vi "Wifi USRP Receiver with Queue.vi"() -> ()   [LabVIEW 2024]
uses:
  <vilib>/Analysis/2dsp.llb/Inverse Complex FFT.vi
  <vilib>/Analysis/2dsp.llb/Complex FFT.vi
  <vilib>/addons/Modulation/Digital/Support/Common/Validators/mod_Validate Number of Rows Columns.vi
  <vilib>/addons/Modulation/Digital/Channel Coding/Block codes/subVIs/mod_Buffer block code info.vi
  <vilib>/addons/Modulation/Digital/DeInterleaving/Block DeInterleaver/mod_Block DeInterleaver (Matrix).vi
  <vilib>/addons/Modulation/Digital/Support/Common/Validators/mod_Generate Bits Validate.vi
  <vilib>/addons/Modulation/Digital/General/subVIs/mod_Generate Bits Pattern.vi
  <vilib>/addons/Modulation/Analog/support/mod_Set Error Source.vi
  <vilib>/addons/Modulation/Digital/General/MT Map PSK Symbols to Bits.vi
  <vilib>/addons/Modulation/Digital/Channel Coding/MT Convolutional Decoder (Viterbi Hard Decision, Rate).vi
  <vilib>/addons/Modulation/Digital/General/MT Map QAM Symbols to Bits.vi
  <vilib>/addons/Modulation/Digital/General/subVIs/mod_Generate Bits PN Sequence.vi
  <instrlib>/niUSRP/niUSRP Fetch Rx Data (CDB).vi
  <vilib>/Analysis/NI_AALPro.lvlib
  <vilib>/addons/Modulation/niDMT.lvlib
panel:
  out "Received Message":string
  out "Fine FO Estimation":dbl(graph)
  out "Coarse FO Estimation":dbl(graph)
  in  "Ts":dbl
  out "Plateau Length":dbl(graph)
  in  "active antenna":string
  in  "gain":dbl format="%#_6f"
  in  "carrier frequency":dbl=100000.0 format="%#_6p"
  in  "IQ rate":dbl=100000.0 format="%#_6p"
  in  "device names":refnum<k15>
  out "Data 2":dbl[](graph)
  out "Data 1":dbl[](graph)
  in  "Stop":bool
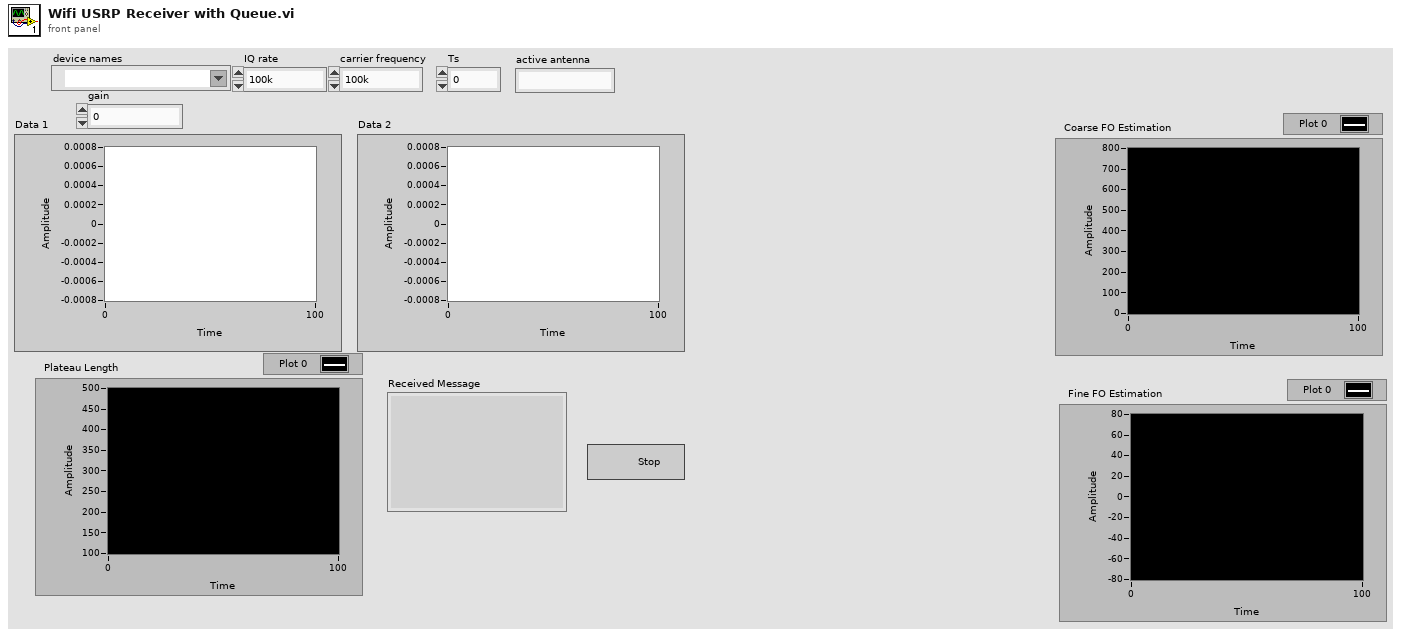
[diagram p1: front panel]
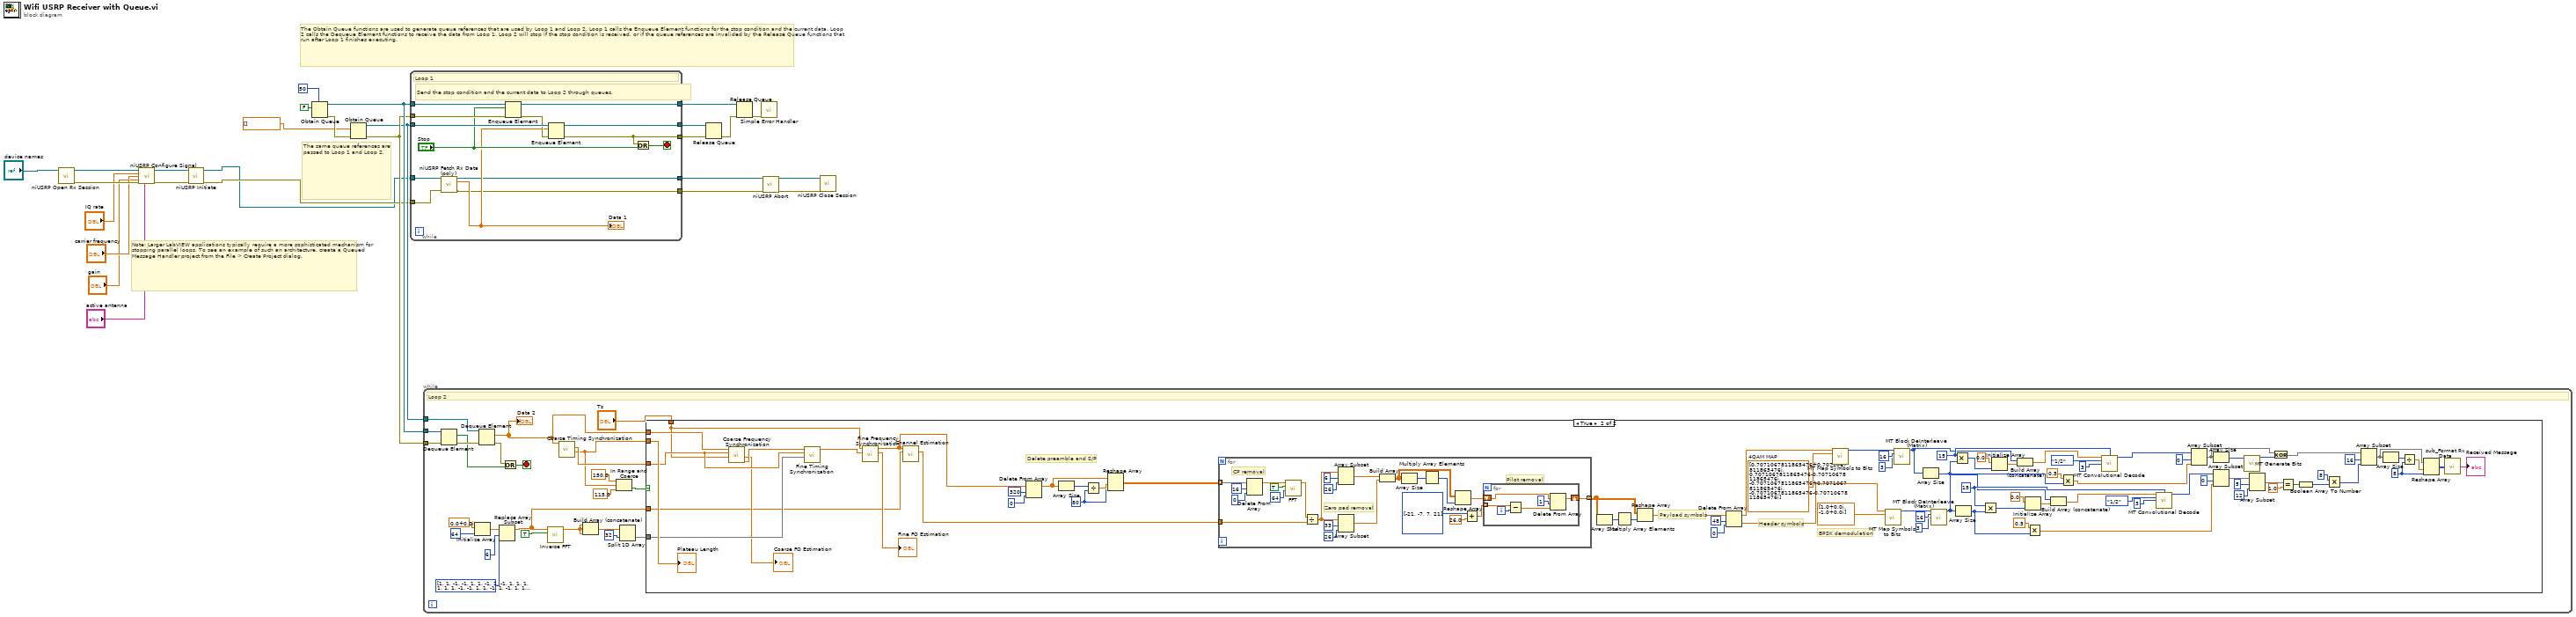
[diagram p0: block diagram]
diagram:
  # "Note: Larger LabVIEW applications typically require a more sophisticated mechanism for stopping parallel loops. To see an example of such an architecture, create a Queued Message Handler project from the File > Create Project dialog."
  # "The same queue references are passed to Loop 1 and Loop 2."
  # "The Obtain Queue functions are used to generate queue references that are used by Loop 1 and Loop 2. Loop 1 calls the Enqueue Element functions for the stop condition and the current data. Loop 2 calls the Dequeue Element functions to receive the data from Loop 1. Loop 2 will stop if the stop condition is received, or if the queue references are invalided by the Release Queue functions that run after Loop 1 finishes executing."
  n1 = call <instrlib>:"niUSRP Open Rx Session.vi"("device names"="device names") -> ("session handle out"=w16:refnum<k15>, "error out"=w14:errorcluster)  [unwired: 13 in]
  n2 = call <instrlib>:"niUSRP Configure Signal.vi"("session handle"=w16, "IQ rate"="IQ rate", "carrier frequency"="carrier frequency", "gain"="gain", "error in (no error)"=w14, "active antenna"="active antenna") -> ("session handle out"=w15:refnum<k15>, "error out"=w13:errorcluster)  [unwired: 5 in, 3 out]
  n3 = call <instrlib>:"niUSRP Initiate.vi"("session handle"=w15, "error in (no error)"=w13) -> ("session handle out"=w6:refnum<k15>, "error out"=w7:errorcluster)  [unwired: 12 in]
  n4 = Obtain Queue(max queue size (-1, unlimited)=50, element data type=FALSE) -> (queue out=w27:refnum<queue>, error out=w25:errorcluster)  [unwired: 3 in, 1 out]
  n5 = Obtain Queue(element data type=cdb[] [], error in (no error)=w25) -> (queue out=w18:refnum<queue>, error out=w19:errorcluster)  [unwired: 3 in, 1 out]
  n6 = while {
    tunnel: w27 -> [w41]
    tunnel: w19 -> [w40]
    tunnel: [w39] -> w21
    tunnel: w18 -> [w38]
    tunnel: [w36] -> w23
    tunnel: [w35] -> w24
    tunnel: w7 -> [w32]
    tunnel: w6 -> [w31]
    tunnel: [w29] -> w3
    tunnel: [w28] -> w2
    stop <- w33 stop-if-true
    # "Send the stop condition and the current data to Loop 2 through queues."
    # "Loop 1"
    n7 = call-poly <instrlib>:"niUSRP Fetch Rx Data (poly).vi"("session handle"=w31, "error in (no error)"=w32) -> ("session handle out"=w28:refnum<k15>, "data"=w30:cdb[], "error out"=w29:errorcluster)  [unwired: 10 in, 1 out]
    "Data 1" <- w30
    n8 = Enqueue Element(queue=w41, element="Stop", error in (no error)=w40) -> (queue out=w39:refnum<queue>, error out=w37:errorcluster)  [unwired: 1 in, 1 out]
    n9 = Enqueue Element(queue=w38, element=w30, error in (no error)=w37) -> (queue out=w36:refnum<queue>, error out=w35:errorcluster)  [unwired: 1 in, 1 out]
    n10 = Or(x=w35, y="Stop") -> (x .or. y?=w33:bool)
  }
  n11 = while {
    tunnel: w27 -> [w65]
    tunnel: w19 -> [w66]
    tunnel: w18 -> [w63]
    stop <- w60 stop-if-true
    # "Loop 2"
    n12 = Dequeue Element(queue=w65, error in (no error)=w66) -> (element=w61:bool, error out=w64:errorcluster)  [unwired: 1 in, 2 out]
    n13 = Initialize Array(cdb 0.0+0.0i ("element"), 64 ("dimension size")) -> (w54:cdb[])
    n14 = Dequeue Element(queue=w63, error in (no error)=w64) -> (element=w57:cdb[], error out=w62:errorcluster)  [unwired: 1 in, 2 out]
    "Data 2" <- w57
    n15 = Replace Array Subset(array=w54, new element=i32[] [1, 1, -1, -1, 1, 1, -1, 1, -1, 1, 1, 1, 1, 1, 1, -1, -1, 1, 1, -1, 1, -1, 1, 1, 1, 1, 0, 1, -1, -1, 1, 1, -1, 1, -1, 1, -1, -1, -1, -1, -1, 1, 1, -1, -1, 1, -1, 1, -1, 1, 1, 1, 1], index=6) -> (w46:cdb[])
    n16 = Or(x=w62, y=w61) -> (x .or. y?=w60:bool)
    n17 = call-poly <vilib>:"Inverse FFT.vi"("shift?"=TRUE ("shift? 3"), "FFT {X}"=w46) -> ("X"=w51:cdb[])  [unwired: 8 in, 1 out]
    n18 = call "Coarse Timing Synchronization.vi"("Array"=w57) -> ("max value"=w45:dbl, "Coarse packet est"=w58:dbl)  [unwired: 9 in]
    n19 = Build Array (concatenate)(w51, w51, w51) -> (w50:cdb[])
    n20 = In Range and Coerce(upper limit=150.0, x=w45, lower limit=115.0 ("y")) -> (In Range?=w42:bool)  [unwired: 1 out]
    n21 = Split 1D Array(array=w50, index=32) -> (second subarray=w47:cdb[])  [unwired: 1 out]
    n22 = case shown="True" w42 {
      tunnel: w45 -> [_ w147]
      tunnel: "Ts" -> [_ w141]
      tunnel: w58 -> [_ w144]
      tunnel: w57 -> [_ w146]
      tunnel: w47 -> [_ w143]
      tunnel: w46 -> [_ w138]
      frame False {
      }
      frame True {
        w73 = 80 ("dimension size")
        w78 = 8 ("y")
        w108 = 15 ("traceback depth (D)")
        w112 = cdb[] [0.7071067811865476+0.7071067811865476i, 0.7071067811865476-0.7071067811865476i, -0.7071067811865476+0.7071067811865476i, -0.7071067811865476-0.7071067811865476i]  # 4QAM MAP
        w120 = 15 ("traceback depth (D)")
        # "Delete preamble and S/P"
        # "Header symbols"
        # "BPSK demodulation"
        # "Payload symbols"
        n23 = call "Coarse Frequency Synchronization.vi"("Ts"=w141, "Numeric in"=w144, "Array in"=w146) -> ("Array out"=w145:cdb[], "coarse freq est"=→"Coarse FO Estimation":dbl)  [unwired: 7 in]
        n24 = call "Fine Timing Synchronization.vi"("Long Preamble"=w143, "Coarse packet est"=w144, "Frame after coarse freq sync"=w145) -> ("Frame after fine time sync"=w140:cdb[])  [unwired: 7 in, 1 out]
        n25 = call "Fine Frequency Synchronization.vi"("Frame after fine time sync"=w140, "Ts"=w141) -> ("Fine freq est"=→"Fine FO Estimation":dbl, "Frame after fine freq sync"=w67:cdb[])  [unwired: 8 in]
        n26 = call "Channel Estimation.vi"("Half of LLTF"=w138, "Frame after fine freq sync in"=w67) -> ("Channel Estimate"=w68:cdb[])  [unwired: 9 in]
        n27 = Delete From Array(array=w67, length=320, index=0) -> (array with subset deleted=w75:cdb[])  [unwired: 1 out]
        n28 = Array Size(array=w75) -> (size(s)=w72:i32)
        n29 = Divide(x=w72, y=w73) -> (x/y=w74:dbl)
        n30 = Reshape Array(w75, w74, w73) -> (w69:cdb[][])
        n31 = for {
          tunnel: w69 -> [w151] mode=indexing
          tunnel: [w153] -> w136 mode=indexing
          tunnel: w68 -> [w150]
          # "Zero pad removal"
          # "Pilot removal"
          # "CP removal"
          n32 = Delete From Array(array=w151, length=16, index=0) -> (array with subset deleted=w167:cdb[])  [unwired: 1 out]
          n33 = call-poly <vilib>:"FFT.vi"("FFT size"=64, "shift?"=TRUE, "X"=w167) -> ("FFT {X}"=w149:cdb[])  [unwired: 7 in, 1 out]
          n34 = Divide(x=w149, y=w150) -> (x/y=w148:cdb[])
          n35 = Array Subset(array=w148, index=6, length=26) -> (w161:cdb[])
          n36 = Array Subset(array=w148, index=33, length=26) -> (w162:cdb[])
          n37 = Build Array(w161, w162) -> (w156:cdb[][])
          n38 = Array Size(array=w156) -> (size(s)=w158:i32[])
          n39 = Multiply Array Elements(1:w158) -> (0:w157:i32)
          n40 = Reshape Array(w156, w157) -> (w154:cdb[])
          n41 = Add(x=i32[] [-21, -7, 7, 21], y=26.0) -> (x+y=w155:dbl[])
          n42 = for {
            tunnel: w155 -> [w175] mode=indexing
            shift-right: [w172] -> w153
            shift-left: w154 -> [w171]
            i -> [w173]
            n43 = Subtract(x=w175, y=w173) -> (x-y=w174:dbl)
            n44 = Delete From Array(array=w171, length=1, index=w174) -> (array with subset deleted=w172:cdb[])  [unwired: 1 out]
          }
        }
        n45 = Array Size(array=w136) -> (size(s)=w137:i32[])
        n46 = Multiply Array Elements(1:w137) -> (0:w135:i32)
        n47 = Reshape Array(w136, w135) -> (w90:cdb[])
        n48 = Delete From Array(array=w90, length=48, index=0) -> (deleted portion=w123:cdb[], array with subset deleted=w89:cdb[])
        n49 = call-poly <vilib>:"MT Map Symbols to Bits.vi"("symbols"=w89, "symbol map"=w112) -> ("output bit stream"=w88:i8[])  [unwired: 12 in, 1 out]
        n50 = call-poly <vilib>:"MT Map Symbols to Bits.vi"("symbols"=w123, "symbol map"=cdb[] [1.0+0.0i, -1.0+0.0i]) -> ("output bit stream"=w129:i8[])  [unwired: 12 in, 1 out]
        n51 = call <vilib>:"MT Block DeInterleave (Matrix).vi"("data in"=w88, "number of rows"=16, "number of columns"=3) -> ("data out"=w104:i32[])  [unwired: 11 in, 1 out]
        n52 = Array Size(array=w104) -> (size(s)=w96:i32)
        n53 = call <vilib>:"MT Block DeInterleave (Matrix).vi"("data in"=w129, "number of rows"=16, "number of columns"=3) -> ("data out"=w113:i32[])  [unwired: 11 in, 1 out]
        n54 = Multiply(x=w108, y=w96) -> (x*y=w109:i32)
        n55 = Array Size(array=w113) -> (size(s)=w93:i32)
        n56 = Multiply(x=w120, y=w93) -> (x*y=w121:i32)
        n57 = Initialize Array(0.0 ("element"), w109) -> (w106:dbl[])
        n58 = Build Array (concatenate)(w104, w106) -> (w105:dbl[])
        n59 = Initialize Array(0.0 ("element"), w121) -> (w118:dbl[])
        n60 = Multiply(x=0.5, y=w93) -> (x*y=w100:dbl)
        n61 = Build Array (concatenate)(w113, w118) -> (w117:dbl[])
        n62 = Multiply(x=0.5, y=w96) -> (x*y=w95:dbl)
        n63 = call-poly <vilib>:"MT Convolutional Decode.vi"("input bit stream"=w105, "traceback depth (D)"=w108, "rate (k/n)"=enum16{"1/2", "1/3", "1/4", "2/3", "3/4"}."1/2", "constraint length (K)"=3) -> ("output bit stream"=w102:i8[])  [unwired: 9 in, 2 out]
        n64 = call-poly <vilib>:"MT Convolutional Decode.vi"("input bit stream"=w117, "traceback depth (D)"=w120, "rate (k/n)"=enum16{"1/2", "1/3", "1/4", "2/3", "3/4"}."1/2", "constraint length (K)"=3) -> ("output bit stream"=w116:i8[])  [unwired: 9 in, 2 out]
        n65 = Array Subset(array=w102, index=0, length=w95) -> (w85:i8[])
        n66 = Array Size(array=w85) -> (size(s)=w87:i32)
        n67 = Array Subset(array=w116, index=0, length=w100) -> (w114:i8[])
        n68 = call <vilib>:"MT Generate Bits.vi"("total bits (128)"=w87) -> ("output bit stream"=w86:i8[])  [unwired: 12 in, 2 out]
        n69 = Array Subset(array=w114, index=5, length=12) -> (w124:i8[])
        n70 = Exclusive Or(1:w86, 2:w85) -> (0:w84:i8[])
        n71 = Equal?(x=w124, y=1.0) -> (x = y?=w125:bool[])
        n72 = Boolean Array To Number(Boolean array=w125) -> (number=w92:u32)
        n73 = Multiply(x=u32 8, y=w92) -> (x*y=w82:u32)
        n74 = Array Subset(array=w84, index=16, length=w82) -> (w81:i8[])
        n75 = Array Size(array=w81) -> (size(s)=w80:i32)
        n76 = Divide(x=w80, y=w78) -> (x/y=w79:dbl)
        n77 = Reshape Array(w81, w79, w78) -> (w77:i8[][])
        n78 = call "sub_Format Rx Data.vi"("Output Packet Array"=w77) -> ("Received Message"=→"Received Message":string)
        "Plateau Length" <- w147
      }
    }
  }
  n79 = Release Queue(queue=w23, error in (no error)=w24) -> (error out=w22:errorcluster)  [unwired: 1 in, 2 out]
  n80 = Release Queue(queue=w21, error in (no error)=w22) -> (error out=w20:errorcluster)  [unwired: 1 in, 2 out]
  n81 = call <vilib>:"Simple Error Handler.vi"("error in (no error)"=w20) -> ()  [unwired: 4 in, 5 out]
  n82 = call <instrlib>:"niUSRP Abort.vi"("session handle"=w2, "error in (no error)"=w3) -> ("session handle out"=w5:refnum<k15>, "error out"=w4:errorcluster)  [unwired: 12 in]
  n83 = call <instrlib>:"niUSRP Close Session.vi"("session handle"=w5, "error in (no error)"=w4) -> ()  [unwired: 13 in, 1 out]
